vi "Drop Protobuf To Field Converter SubVI.vi"(8 "error in (no error)":errorcluster, 10 "Owner VI in":refnum<vi>, 11 "Library":refnum<vi>) -> (0 "error out":errorcluster, 1 "SubVI out":refnum<vi>, 2 "Owner VI out":refnum<vi>, 3 "Library out":refnum<vi>)   [LabVIEW 2019, in "gRPC Template Creation Utility.lvlib"]
uses:
  gRPC Template Creation Utility.lvlib
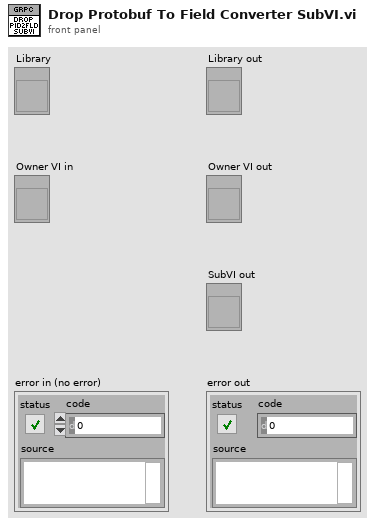
[diagram p1: front panel]
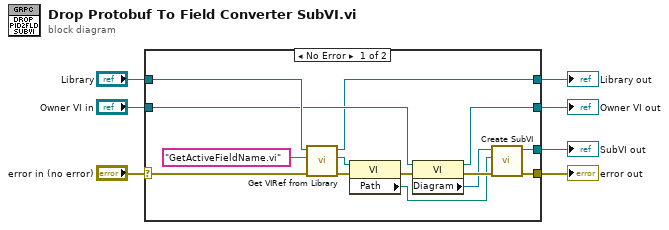
[diagram p0: block diagram]
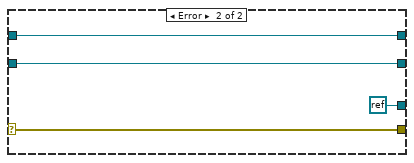
[diagram p2: hidden frame]
diagram:
  n1 = case shown="No Error" "error in (no error)" {
    selector: "error in (no error)" -> [w10 w25]
    tunnel: [w21 refnum<k0> refnum] -> w7
    tunnel: [w20 w25] -> w6
    tunnel: "Library" -> [w14 w24]
    tunnel: "Owner VI in" -> [w12 w22]
    tunnel: [w11 w22] -> w3
    tunnel: [w9 w24] -> w1
    frame No Error {
      n2 = call "Get VIRef from Library.vi"("error in (no error)"=w10, "item name"="GetActiveFieldName.vi" ("format string"), "library in"=w14) -> ("error out"=w16:errorcluster, "vi"=w15:refnum<vi>, "library out"=w9:refnum<vi>)  [unwired: 5 in, 1 out]
      n3 = property class="VI"(reference=w15, error in=w16) -> (error out=w18:errorcluster, "Path"=w17:path)  [unwired: 1 out]
      n4 = property class="VI"(reference=w12, error in=w18) -> (reference out=w11:refnum<vi>, error out=w19:errorcluster, "Diagram"=w13:refnum<vi>)
      n5 = call "Create SubVI.vi"("error in (no error)"=w19, "Path"=w17, "Diagram in"=w13) -> ("error out"=w20:errorcluster, "subVI refnum"=w21:refnum<vi>)  [unwired: 7 in]
    }
    frame Error {
    }
  }
  "SubVI out" <- w7
  "error out" <- w6
  "Library out" <- w1
  "Owner VI out" <- w3
